vi "RemoteVI Refresh Geometry.vi"(0 "VI":refnum<vi>, 1 "now":u32, 2 "geometry due?":bool, 3 "popup was open?":bool, 5 "geo":T1, 7 "hWnd":u64, 9 "last refresh":u32, 11 "origin":cluster{"x":i32, "y":i32}, 12 "popup open?":bool, 13 "recent click?":bool, 14 "window":u64) -> (4 "geo out":T1, 6 "hWnd out":u64, 8 "last refresh out":u32, 10 "origin out":cluster{"x":i32, "y":i32})   [LabVIEW 2020, in "RemoteVI.lvlib"]
doc: "Refreshes the server loop's cached panel geometry, window handle and panel origin inside the frame (RemoteVI Get Panel Geometry.vi - a VI Server call) when it is due - 500 ms after the last refresh (geometry due?) or right after the last popup closed - but only while NO popup is open and not within 300 ms of a click (recent click?); on an error the cached values are kept. last refresh out is now after a refresh, else last refresh."
uses:
  RemoteVI.lvlib
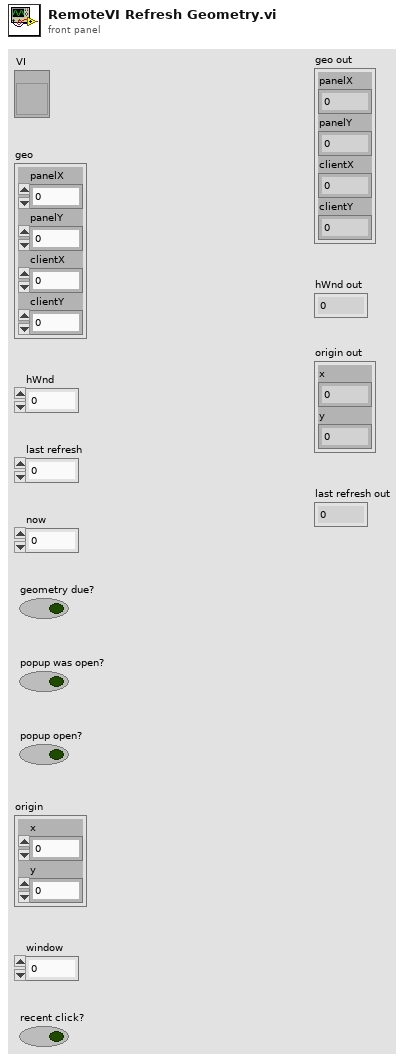
[diagram p1: front panel]
types:
  T1 = cluster{"panelX":i32, "panelY":i32, "clientX":i32, "clientY":i32}
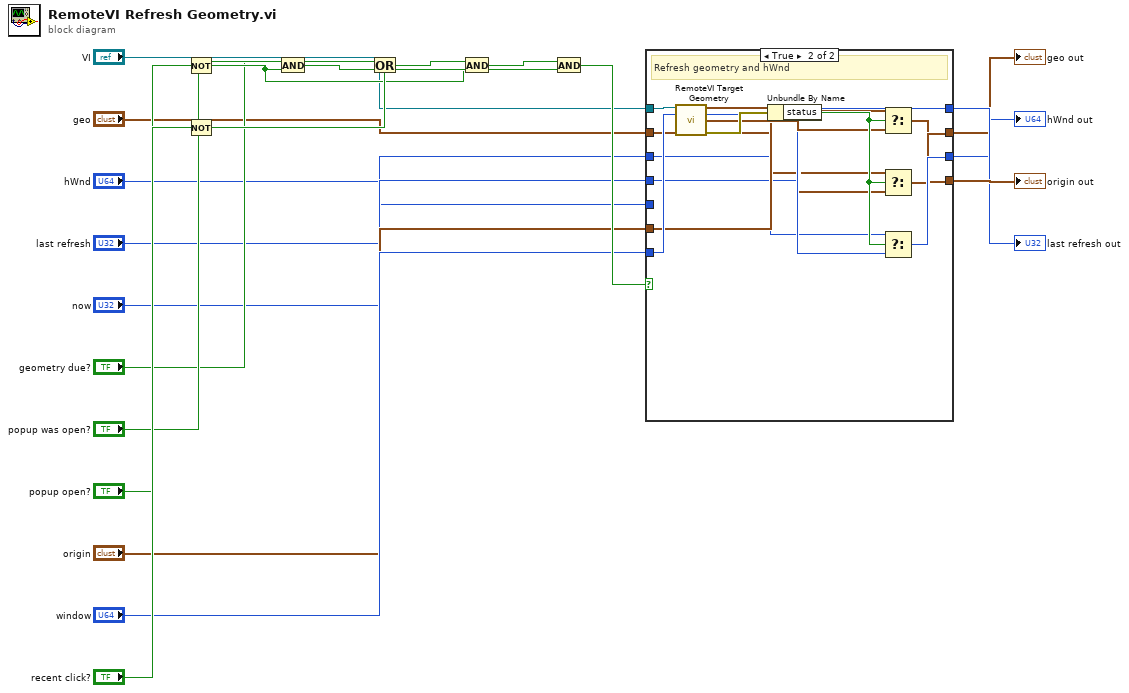
[diagram p0: block diagram]
diagram:
  n1 = Not(x="popup open?") -> (.not. x?=w12:bool)
  n2 = Not(x="recent click?") -> (.not. x?=w15:bool)
  n3 = And(x="popup was open?", y=w12) -> (x .and. y?=w13:bool)
  n4 = Or(x="geometry due?", y=w13) -> (x .or. y?=w14:bool)
  n5 = And(x=w14, y=w12) -> (x .and. y?=w16:bool)
  n6 = And(x=w16, y=w15) -> (x .and. y?=w17:bool)
  n7 = case shown="True" w17 {
    tunnel: "VI" -> [_ w26]
    tunnel: "geo" -> [w22 w27]
    tunnel: "hWnd" -> [w23 w28]
    tunnel: "now" -> [_ w29]
    tunnel: "last refresh" -> [w24 _]
    tunnel: "origin" -> [w25 w30]
    tunnel: "window" -> [_ w31]
    tunnel: [w24 w29] -> w20
    tunnel: [w22 w38] -> w18
    tunnel: [w23 w39] -> w19
    tunnel: [w25 w36] -> w21
    frame False {
    }
    frame True {
      # "Refresh geometry and hWnd"
      n8 = call "RemoteVI Target Geometry.vi"("VI"=w26, "window"=w31) -> ("geo"=w32:T1, "hWnd"=w33:u64, "origin"=w34:cluster{"x":i32, "y":i32}, "error out"=w35:errorcluster)  [unwired: 10 in]
      n9 = Unbundle By Name(w35) -> ("status"=w37:bool)
      n10 = Select(t=w30, s=w37, f=w34) -> (s? t:f=w36:cluster{"x":i32, "y":i32})
      n11 = Select(t=w27, s=w37, f=w32) -> (s? t:f=w38:T1)
      n12 = Select(t=w28, s=w37, f=w33) -> (s? t:f=w39:u64)
    }
  }
  "geo out" <- w18
  "hWnd out" <- w19
  "origin out" <- w21
  "last refresh out" <- w20
